vi "bring_to_initial_position_producerconsumer__d646e2174d.vi"(0 "DAQ in":refnum<k21>, 1 "Initial position in Voltage (V) in":dbl, 5 "SMU error in":errorcluster, 7 "Initial PID gains":T1, 9 "DAQ error in":errorcluster, 11 "SMU in":refnum<k15>) -> (2 "SMUstatus":bool, 3 "position":dbl format="%0.2f", 4 "SMU out":refnum<k15>, 6 "SMU error out":errorcluster, 8 "Boolean":bool, 10 "DAQ error out":errorcluster, 12 "DAQ status":bool, 13 "current":dbl format="%_6g", 14 "votage":dbl caption="voltage" format="%_6g", 15 "DAQ out":refnum<k21>)   [LabVIEW 2023]
uses:
  <instrlib>/niDCPower/nidcpower.llb/niDCPower Measurement Type.ctl
  <vilib>/DAQmx/read.llb/DAQmx Read (Analog DBL 1Chan 1Samp).vi
  <vilib>/DAQmx/miscellaneous.llb/DAQmx Fill In Error Info.vi
  <vilib>/addons/control/pid/pid.llb/PID Advanced (DBL).vi
  <vilib>/addons/control/pid/NI_PID_pid.lvlib
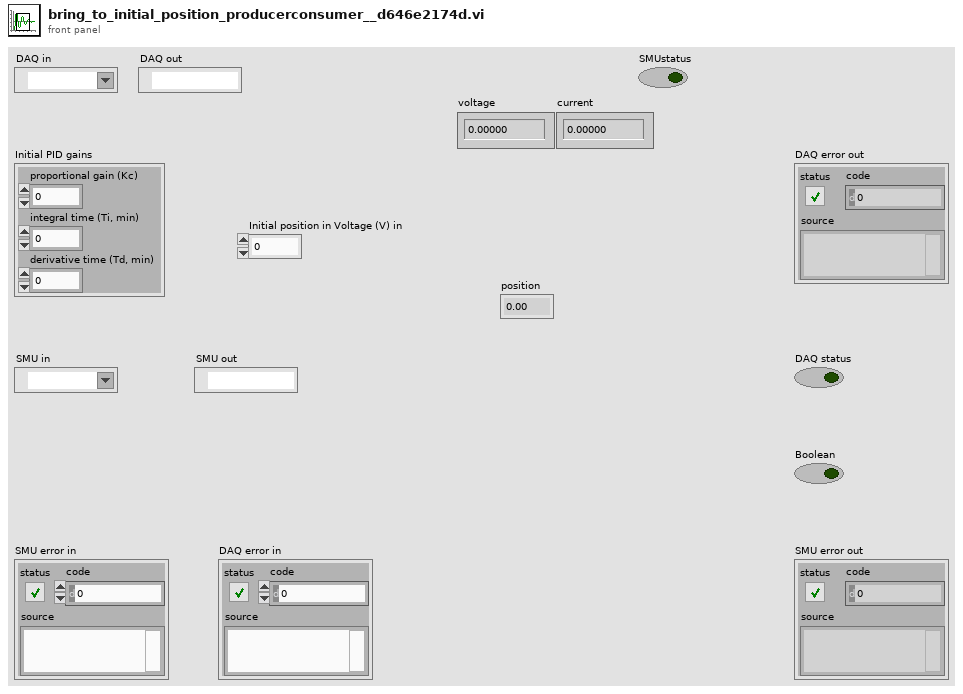
[diagram p1: front panel]
types:
  T1 = cluster{"proportional gain (Kc)":dbl, "integral time (Ti, min)":dbl, "derivative time (Td, min)":dbl}
  T2 = typedef "niDCPower Measurement Type.ctl" = i32
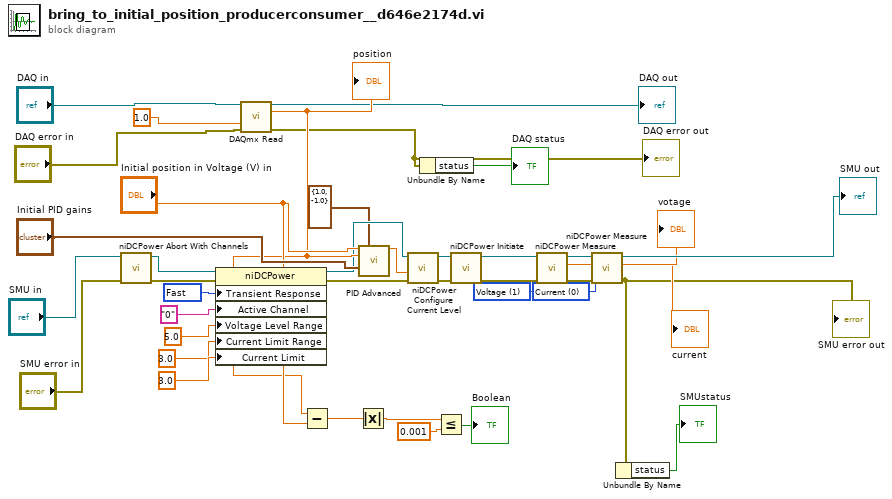
[diagram p0: block diagram]
diagram:
  w5 = T2 0 items=["Current", "Voltage"] ("measurement type")
  w6 = T2 1 items=["Current", "Voltage"] ("measurement type")
  w14 = 1039 items=["Slow"=1041, "Normal"=1038, "Fast"=1039, "Custom"=1042] ("Source:Transient Response")
  n1 = call <instrlib>:"niDCPower Abort With Channels.vi"("error in (no error)"="SMU error in", "instrument handle"="SMU in") -> ("error out"=w19:errorcluster, "instrument handle out"=w18:refnum<k15>)  [unwired: 8 in]
  n2 = property class="niDCPower"(reference=w18, error in=w19, "Transient Response"=w14, "Active Channel"="0", "Voltage Level Range"=5.0 ("Source:DC Voltage:Voltage Level Range"), "Current Limit Range"=3.0 ("Source:DC Voltage:Current Limit Range"), "Current Limit"=3.0 ("Source:DC Voltage:Current Limit")) -> (reference out=w20:refnum<k15>, error out=w21:errorcluster)
  n3 = call-poly <vilib>:"DAQmx Read.vi"("task/channels in"="DAQ in", "timeout"=1.0, "error in"="DAQ error in") -> ("task out"=→"DAQ out":refnum<k21>, "data"=w32:dbl, "error out"=w31:errorcluster)  [unwired: 10 in]
  "DAQ error out" <- w31
  "position" <- w32
  n4 = Subtract(x=w32, y="Initial position in Voltage (V) in") -> (x-y=w28:dbl)
  n5 = Absolute Value(x=w28) -> (abs(x)=w29:dbl)
  n6 = call-poly <vilib>:"PID Advanced.vi"("setpoint"="Initial position in Voltage (V) in", "output range"=cluster{"output high":dbl, "output low":dbl} {"output high"=1.0, "output low"=-1.0}, "process variable"=w32, "PID gains"="Initial PID gains") -> ("output"=w27:dbl)  [unwired: 10 in, 1 out]
  n7 = call <instrlib>:"niDCPower Configure Current Level.vi"("error in (no error)"=w21, "current level"=w27, "instrument handle"=w20) -> ("error out"=w23:errorcluster, "instrument handle out"=w22:refnum<k15>)  [unwired: 7 in]
  n8 = Unbundle By Name(w31) -> ("status"=→"DAQ status":bool)
  n9 = Less Or Equal?(x=w29, y=0.001) -> (x <= y?=→"Boolean":bool)
  n10 = call <instrlib>:"niDCPower Initiate.vi"("error in (no error)"=w23, "instrument handle"=w22) -> ("error out"=w11:errorcluster, "instrument handle out"=w10:refnum<k15>)  [unwired: 2 in, 6 out]
  n11 = call <instrlib>:"niDCPower Measure.vi"("error in (no error)"=w11, "measurement type"=w6, "instrument handle"=w10) -> ("error out"=w7:errorcluster, "measurement"=→"votage":dbl, "instrument handle out"=w9:refnum<k15>)  [unwired: 6 in]
  n12 = call <instrlib>:"niDCPower Measure.vi"("error in (no error)"=w7, "measurement type"=w5, "instrument handle"=w9) -> ("error out"=w2:errorcluster, "measurement"=→"current":dbl, "instrument handle out"=→"SMU out":refnum<k15>)  [unwired: 6 in]
  "SMU error out" <- w2
  n13 = Unbundle By Name(w2) -> ("status"=→"SMUstatus":bool)
